vi "Read packageCount.vi"(8 "error in (no error)":errorcluster, 11 "ZM-HWM-hardware_manager in":refnum<class "ZM-HWM-hardware_manager.lvclass">) -> (0 "error out":errorcluster, 2 "packageCount":u32, 3 "ZM-HWM-hardware_manager out":refnum<class "ZM-HWM-hardware_manager.lvclass">)   [LabVIEW 2020, in "ZM-HWM-hardware_manager.lvlib" / "ZM-HWM-hardware_manager.lvclass"]
doc: "Reads one field of this class's private data. Generated by lvai_create_accessors from the class private data control."
uses:
  ZM-HWM-hardware_manager.lvclass
  ZM-HWM-hardware_manager.lvclass/ZM-HWM-hardware_manager.ctl
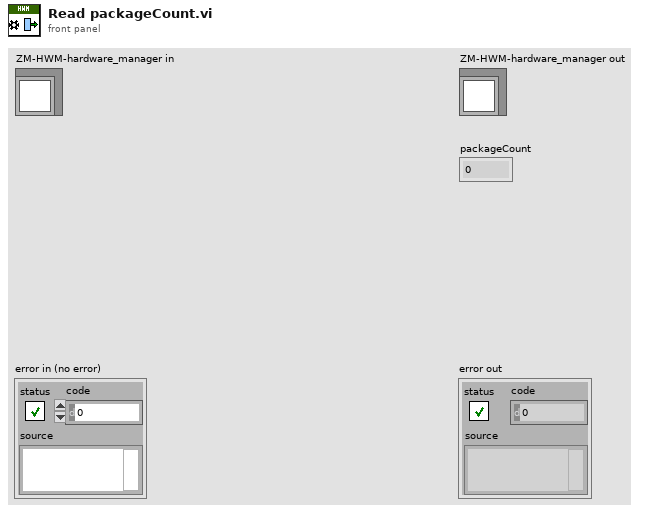
[diagram p1: front panel]
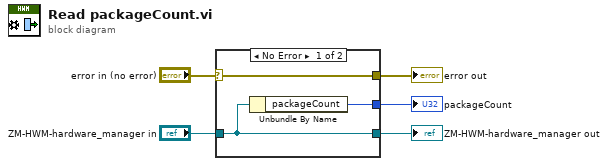
[diagram p0: block diagram]
diagram:
  n1 = case shown="No Error" "error in (no error)" {
    selector: "error in (no error)" -> [w8 w9]
    tunnel: [w8 w9] -> w4
    tunnel: [w7 w10] -> w2
    tunnel: "ZM-HWM-hardware_manager in" -> [w7 w10]
    tunnel: [w6 _] -> w1
    frame No Error {
      n2 = Unbundle By Name(w7) -> ("packageCount"=w6:u32)
    }
    frame Error {
    }
  }
  "error out" <- w4
  "ZM-HWM-hardware_manager out" <- w2
  "packageCount" <- w1
